vi "GetGUID.vi"(8 "error in (no error)":errorcluster, 11 "Link in":refnum<class "Link.lvclass">) -> (0 "error out":errorcluster, 2 "GUID":string, 3 "Link out":refnum<class "Link.lvclass">)   [LabVIEW 2023, in "GettingStartedWindow.lvlib" / "Link.lvclass"]
uses:
  <resource>/modes/FRC/GSW/Classes/Link/Link.lvclass
  <resource>/modes/FRC/GSW/Classes/Link/Link.lvclass/Link.ctl
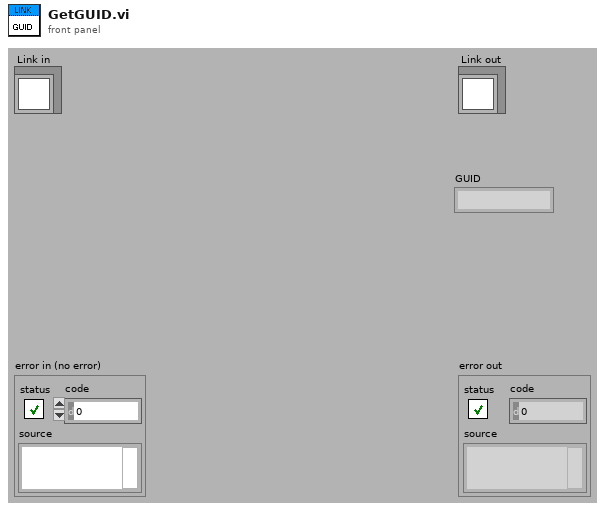
[diagram p1: front panel]
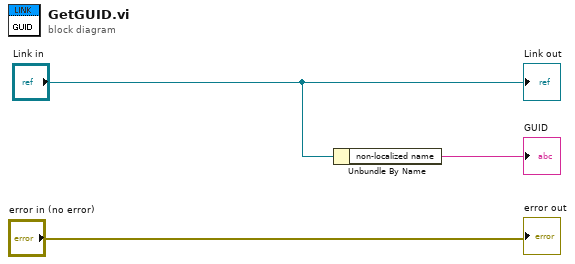
[diagram p0: block diagram]
diagram:
  n1 = Unbundle By Name("Link in") -> ("non-localized name"=→"GUID":string)
  "error out" <- "error in (no error)"
  "Link out" <- "Link in"
